vi "Main.vi"() -> ()   [LabVIEW 2020]
doc: "This template is for the Queued Message Handler design pattern.\n\nThe Event Handling Loop generates messages based on user interface actions.\n\nThe Message Handling Loop processes messages generated by the Event Handling Loop, or by other messages. The messages are string values, so new messages can be added easily to the Message Cases case structure in the Message Handling Loop. Each message cluster can also provide an optional value for Message Data, which is a variant that can be converted to whatever message-specific data is required."
uses:
  <vilib>/ErrorRing/Error Ring.xnode
  controls/oled UI Data.ctl
  support/Message Queue/oled Message Queue.lvlib
  support/User Event - Stop/oled User Event - Stop.lvlib
  support/Message Queue/Enqueue Message (Single).vi
  controls/HL Acq Data.ctl
  controls/Acquisition data --typedef.ctl
  controls/Graph data --typedef.ctl
  <vilib>/Utility/error.llb/Error Cluster From Error Code.vi
  <vilib>/DAQmx/read.llb/DAQmx Read (Analog DBL 1Chan 1Samp).vi
  <vilib>/Instr/_visa.llb/VISA Configure Serial Port (Instr).vi
  <vilib>/DAQmx/create/channels.llb/DAQmx Create Channel (AI-Voltage-Basic).vi
  support/Message Queue/Enqueue Message (Array).vi
  controls/Color --typedef.ctl
panel:
  in  "Color":T1 caption="Color de emisión"
  in  "Inicio de Barrido (V)":dbl
  out "Status":string
  in  "milliseconds to wait":i32=200
  out "Eff L-V":cluster{dbl[], dbl[]}(graph) caption="L-V"
  out "EFf I-V":cluster{dbl[], dbl[]}(graph) caption="L-V"
  in  "Puerto serial Fuente":refnum<visa-resource-name>="COM1"
  out "J-V":cluster{dbl[], dbl[]}(graph)
  out "L-V":cluster{dbl[], dbl[]}(graph)
  in  "OLED A":dbl=0.07 caption="Area del OLED [cm2]"
  in  "OLED-PD dist":dbl=1.0 caption="Distancia OLED-fotodiodo [cm]"
  in  "Protection C":dbl=0.1 caption="Corriente de Proteccion [A]\n(0.1-0.3A recomendado)"
  in  "Max V":dbl=2.0 caption="Voltaje máximo [V]\n(20V max. recomendado)"
  in  "Iniciar":bool
  in  "Step #":dbl=100.0 caption="Numero de pasos\n(100-250 recomendado)"
  in  "Exit":bool
  # "Sistema de caracterización de OLEDs"
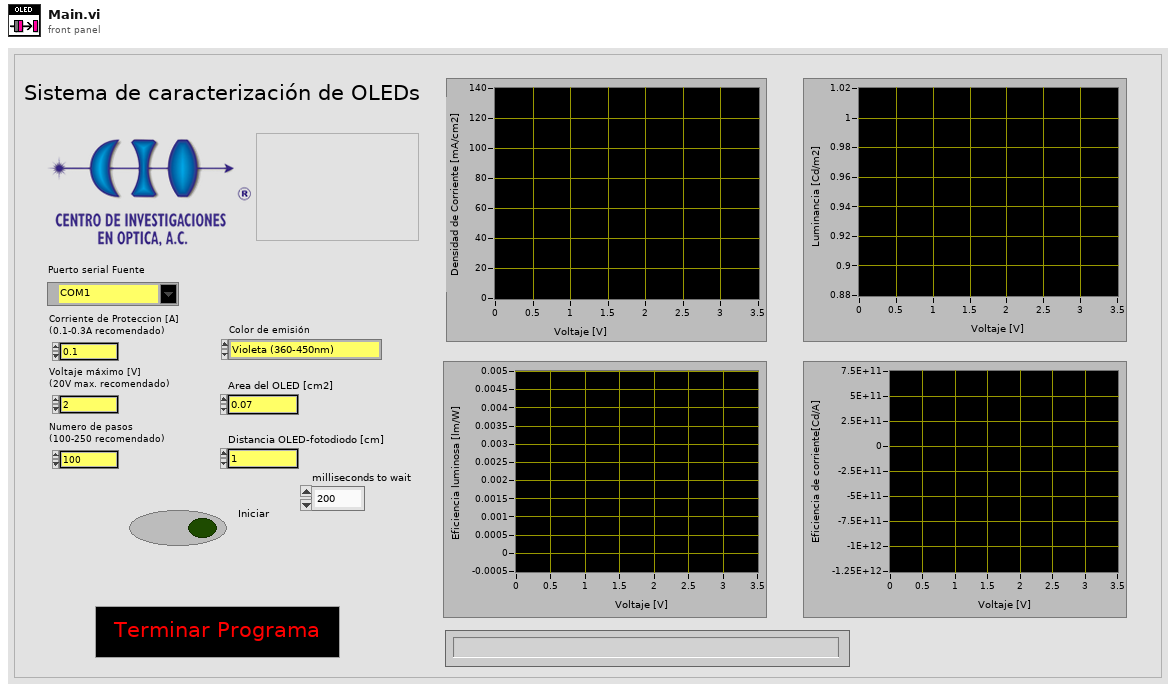
[diagram p1: front panel]
types:
  T1 = typedef "Color --typedef.ctl" = enum16{"Violeta (360-450nm)", "Azul (450-500nm)", "Verde(500-570nm)", "Amarillo (570-590nm)", "Naranja (600-610nm)", "Rojo (610-670nm)", "Blanco"}
  T2 = typedef "oled UI Data.ctl" = cluster{"Status":string, "Puerto serial":refnum<visa-resource-name>, "AI task":refnum<k21>, "Protection C":dbl, "Sweep start V":dbl, "Max V":dbl, "delta V":dbl, "Graph data":T3}
  T3 = typedef "Graph data --typedef.ctl" = cluster{"Voltaje [V]":dbl[], "Corriente [mA]":dbl[], "Densidad de corriente [CD/A]":dbl[], "Iluminancia [Lm/m2]":dbl[], "Luminance [Cd/m2]":dbl[], "Ef corriente [Cd/A]":dbl[], "Ef Luminosa [Cd/W]":dbl[], "V detector [V]":dbl[], "Pin [W]":dbl[]}
  T4 = cluster{"User event - Stop":refnum<user-event>, "User event - Sleep HL":refnum<user-event>, "User event -  Wake HL":refnum<user-event>}
  T5 = typedef "oled Message Queue.lvlib/All Message Queues.ctl" = cluster{"UI":refnum<queue>}
  T6 = typedef "HL Acq Data.ctl" = cluster{"dV":dbl, "Vmax":dbl, "Vo":dbl}
  T7 = typedef "Acquisition data --typedef.ctl" = cluster{"Iluminancia  lm/m2":dbl, "DAQ AV":dbl, "Luminancia (Cd/m2)":dbl, "Pin(W)":dbl, "SM V":dbl, "SM I":dbl, "OLED Area cm2":dbl}
  T8 = cluster{"Voltaje [V]":dbl[], "Luminance [Cd/m2]":dbl[]}
  T9 = cluster{"Voltaje [V]":dbl[], "V detector [V]":dbl[]}
  T10 = cluster{"Voltaje [V]":dbl[], "Ef corriente [Cd/A]":dbl[]}
  T11 = cluster{"Voltaje [V]":dbl[], "Corriente [mA]":dbl[]}
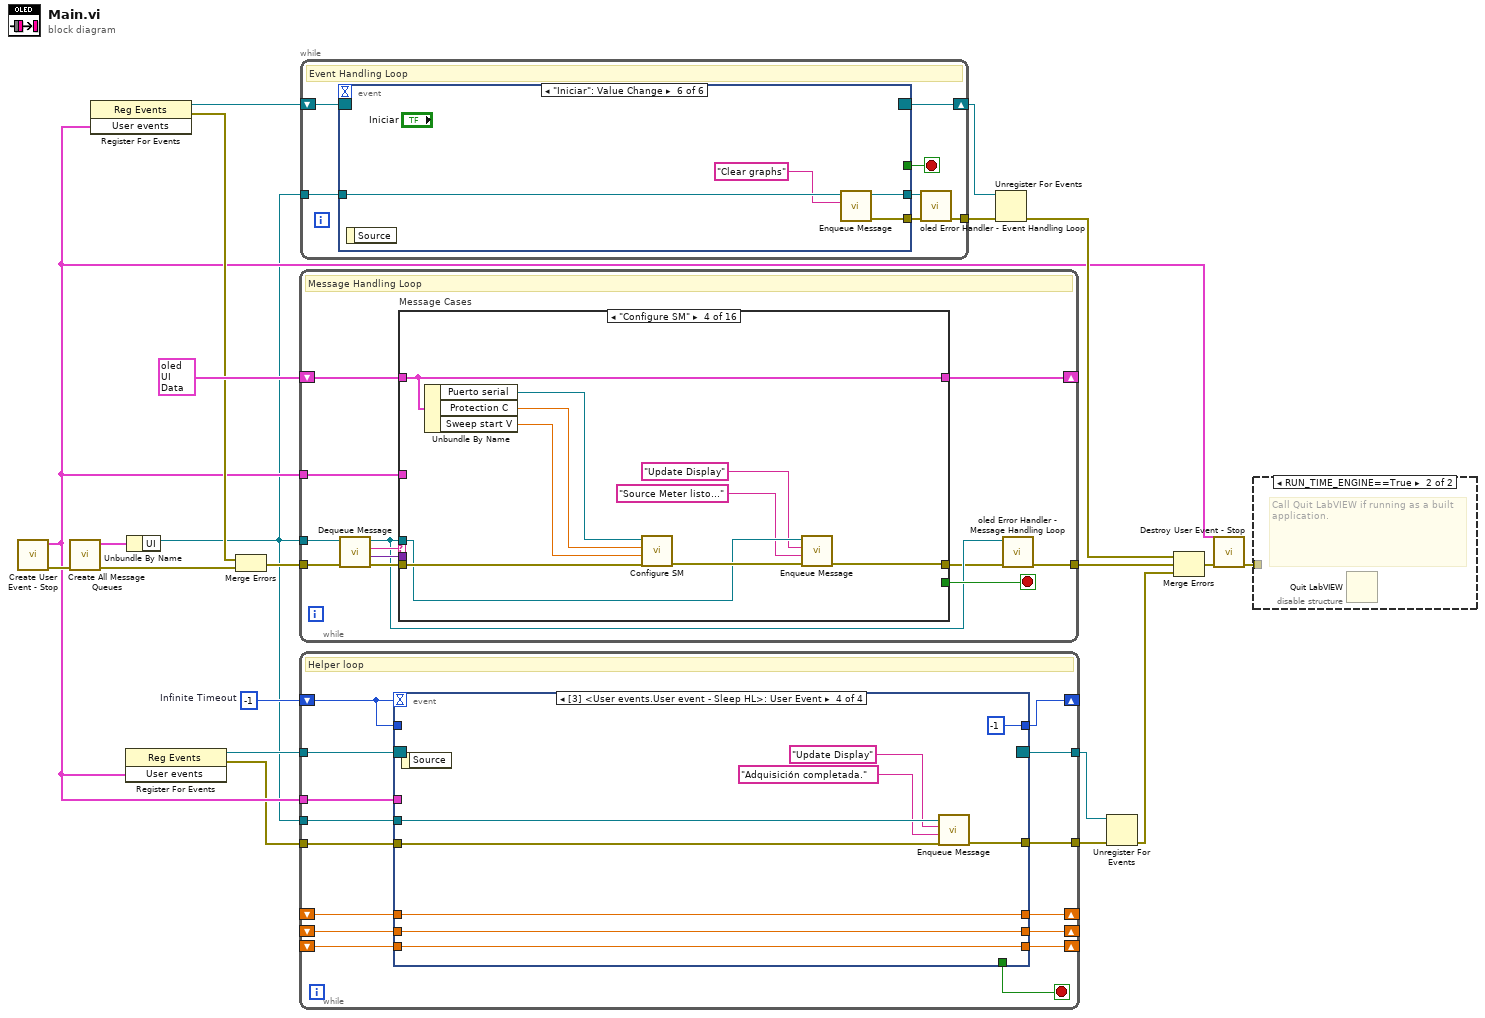
[diagram p0: block diagram]
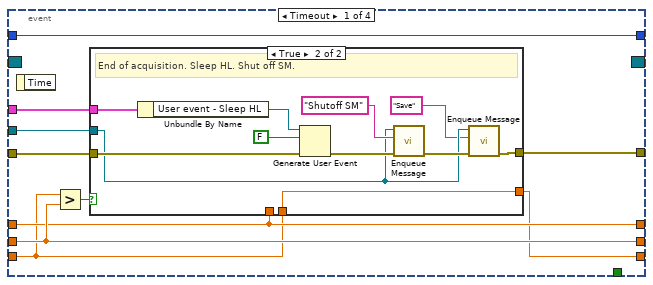
[diagram p2: hidden frame]
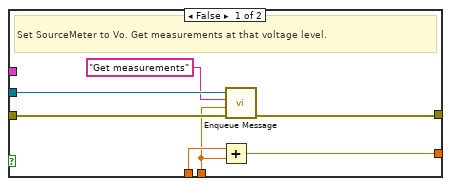
[diagram p3: hidden frame]
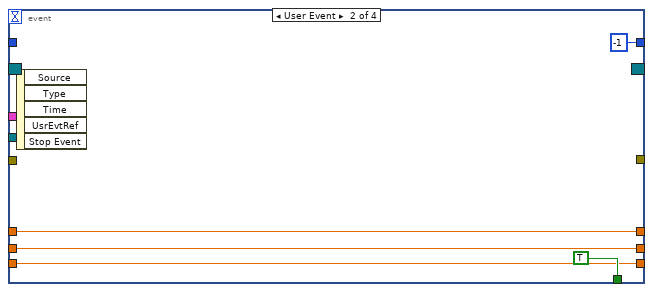
[diagram p4: hidden frame]
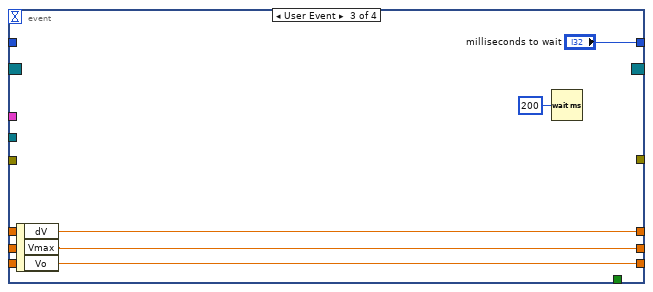
[diagram p5: hidden frame]
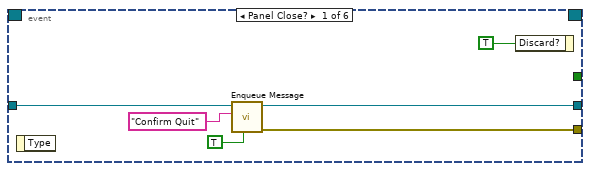
[diagram p6: hidden frame]
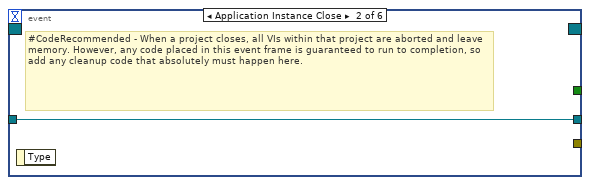
[diagram p7: hidden frame]
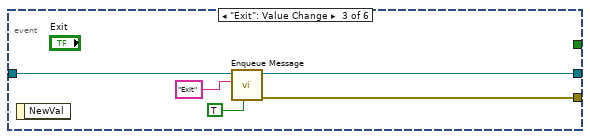
[diagram p8: hidden frame]
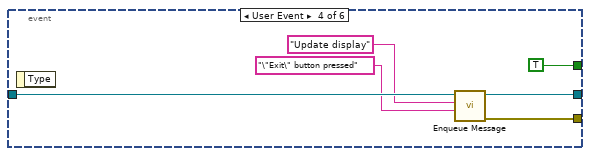
[diagram p9: hidden frame]
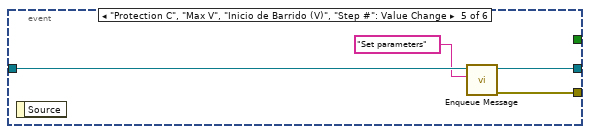
[diagram p10: hidden frame]
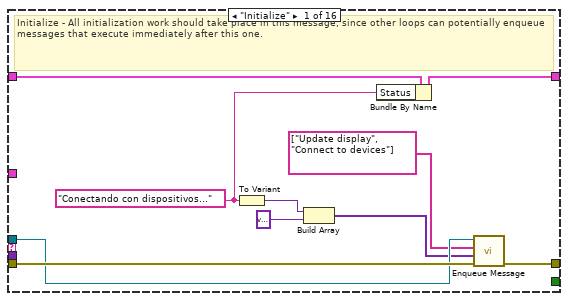
[diagram p11: hidden frame]
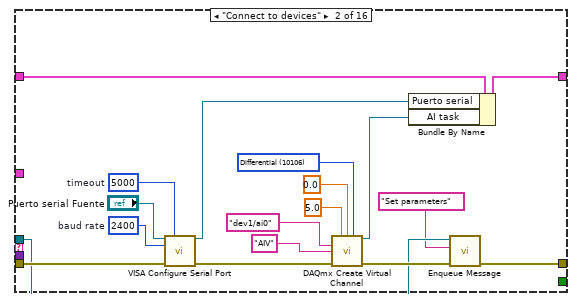
[diagram p12: hidden frame]
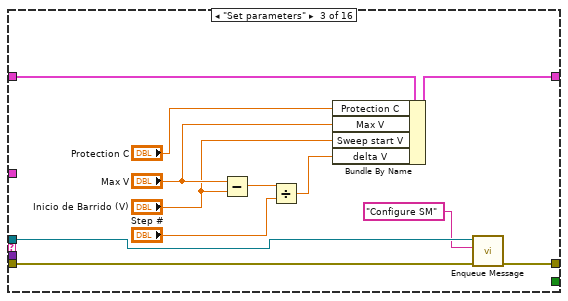
[diagram p13: hidden frame]
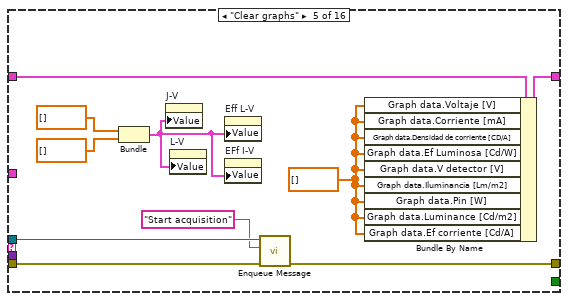
[diagram p14: hidden frame]
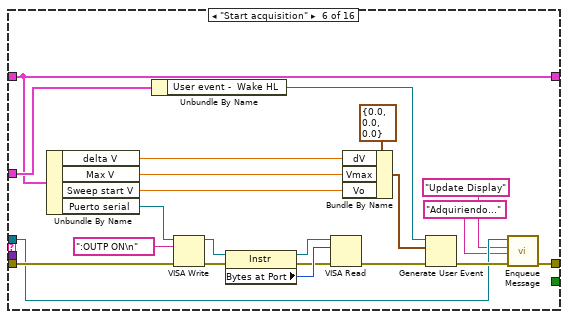
[diagram p15: hidden frame]
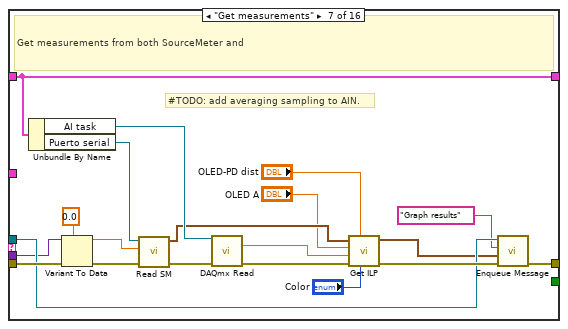
[diagram p16: hidden frame]
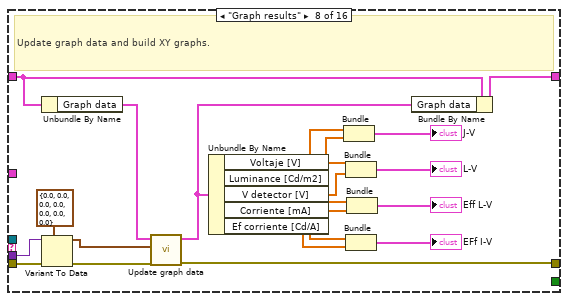
[diagram p17: hidden frame]
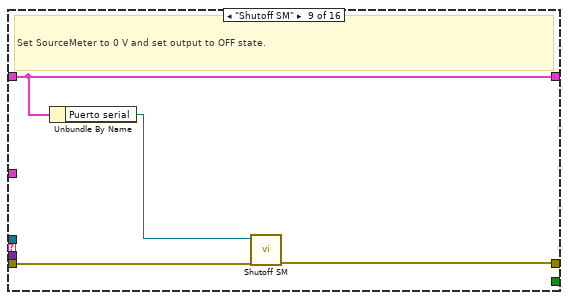
[diagram p18: hidden frame]
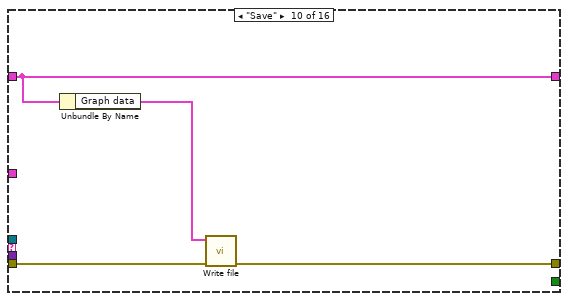
[diagram p19: hidden frame]
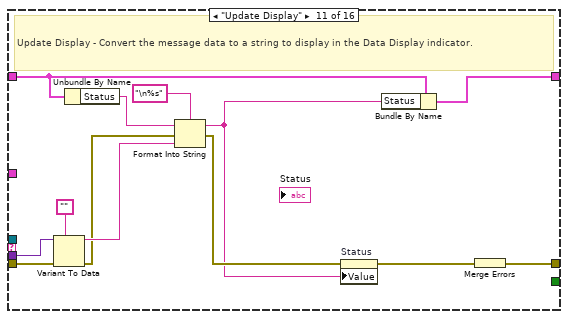
[diagram p20: hidden frame]
diagram:
  w9 = -1  # Infinite Timeout
  n1 = call "Create User Event - Stop.vi"() -> ("error out"=w19:errorcluster, "User events"=w4:T4)  [unwired: 10 in]
  n2 = call "Create All Message Queues.vi"("error in (no error)"=w19) -> ("error out"=w21:errorcluster, "Message Queues out"=w20:T5)  [unwired: 9 in]
  n3 = register-events(w4) -> (reference out=w12:refnum<event-registration>, error out=w10:errorcluster)  [unwired: 2 in]
  n4 = register-events(w4) -> (reference out=w8:refnum<event-registration>, error out=w2:errorcluster)  [unwired: 2 in]
  n5 = Unbundle By Name(w20) -> ("UI"=w1:refnum<queue>)
  n6 = Merge Errors(w10, w21) -> (w11:errorcluster)
  n7 = while {
    tunnel: w1 -> [w25]
    shift-right: [w32] -> _
    shift-left: T2 {"Status"="", "Puerto serial"="", "AI task"="", "Protection C"=0.0, "Sweep start V"=0.0, "Max V"=0.0, "delta V"=0.0, "Graph data"={"Voltaje [V]"=[], "Corriente [mA]"=[], "Densidad de corriente [CD/A]"=[], "Iluminancia [Lm/m2]"=[], "Luminance [Cd/m2]"=[], "Ef corriente [Cd/A]"=[], "Ef Luminosa [Cd/W]"=[], "V detector [V]"=[], "Pin [W]"=[]}} ("Data Cluster") -> [w33]
    tunnel: w4 -> [w30]
    tunnel: w11 -> [w29]
    tunnel: [w23] -> w6
    stop <- w31 stop-if-true
    # "Message Handling Loop"
    n8 = call "Dequeue Message.vi"("error in (no error)"=w29, "Message Queue"=w25) -> ("error out"=w28:errorcluster, "Message Data"=w26:variant, "Message"=w27:string, "dup Message Queue"=w24:refnum<queue>)  [unwired: 6 in]
    n9 = case "Message Cases" shown="\"Configure SM\"" w27 {
      selector: w27 -> [_ _ _ _ _ _ _ _ _ _ _ _ _ _ _ w223]
      tunnel: w24 -> [w39 w45 w63 w76 w85 w104 w127 _ _ _ _ w176 w192 _ w222 _]
      tunnel: w28 -> [w42 w61 w65 w79 w87 w110 w135 w154 w158 w160 w174 w184 w196 w199 w216 _]
      tunnel: [w43 w46 w64 w77 w86 w105 w128 w146 w157 w159 w175 w179 w194 w197 w219 w224] -> w22
      tunnel: w33 -> [w41 w57 w72 w83 w88 w108 w134 w149 w156 w162 w165 w183 w195 w198 w212 w225]
      tunnel: [w40 w55 w67 w83 w90 w108 w134 w148 w156 w162 w163 w183 w195 w198 w212 w225] -> w32
      tunnel: [_ _ _ _ _ _ _ _ _ _ _ _ _ _ TRUE _] -> w31
      tunnel: w26 -> [_ _ _ _ _ _ w118 w152 _ _ w173 w182 _ _ w213 _]
      tunnel: w30 -> [_ _ _ _ _ w111 _ _ _ _ _ _ _ _ w218 _]
      frame "Initialize" {
        w34 = "Conectando con dispositivos..." ("Initial Message")
        # "Initialize - All initialization work should take place in this message, since other loops can potentially enqueue messages that execute immediately after this one."
        n10 = To Variant(anything=w34) -> (Variant=w37:variant)
        n11 = Build Array(w37, variant ("element")) -> (w35:variant[])
        n12 = Bundle By Name(cluster=w41, "Status"=w34) -> (w40:T2)
        n13 = call-poly "Enqueue Message.vi"("error in (no error)"=w42, "Message Data Array"=w35, "Message Array"=string[] ["Update display", "Connect to devices"] ("Message"), "Message Queue"=w39) -> ("error out"=w43:errorcluster)  [unwired: 6 in, 1 out]
      }
      frame "Connect to devices" {
        w49 = 10106 items=["Default"=-1, "RSE"=10083, "NRSE"=10078, "Differential"=10106, "Pseudodifferential"=12529] ("input terminal configuration")
        w58 = u32 5000  # timeout
        w59 = u32 2400  # baud rate
        n14 = call-poly "VISA Configure Serial Port"("VISA resource name"="Puerto serial Fuente", "timeout (10sec)"=w58, "baud rate (9600)"=w59, "error in (no error)"=w61) -> ("VISA resource name out"=w56:refnum<visa-resource-name>, "error out"=w54:errorcluster)  [unwired: 3 in, 7 out]
        n15 = call-poly <vilib>:"DAQmx Create Virtual Channel.vi"("maximum value"=5.0, "minimum value"=0.0, "input terminal configuration"=w49, "physical channels"="dev1/ai0", "name to assign"="AIV", "error in"=w54) -> ("task out"=w48:refnum<k21>, "error out"=w47:errorcluster)  [unwired: 8 in]
        n16 = Bundle By Name(cluster=w57, "Puerto serial"=w56, "AI task"=w48) -> (w55:T2)
        n17 = call-poly "Enqueue Message.vi"("error in (no error)"=w47, "Message"="Set parameters", "Message Queue"=w45) -> ("error out"=w46:errorcluster)  [unwired: 7 in, 1 out]
      }
      frame "Set parameters" {
        n18 = Subtract(x="Max V", y="Inicio de Barrido (V)") -> (x-y=w73:dbl)
        n19 = Divide(x=w73, y="Step #") -> (x/y=w68:dbl)
        n20 = Bundle By Name(cluster=w72, "Protection C"="Protection C", "Max V"="Max V", "Sweep start V"="Inicio de Barrido (V)", "delta V"=w68) -> (w67:T2)
        n21 = call-poly "Enqueue Message.vi"("error in (no error)"=w65, "Message"="Configure SM", "Message Queue"=w63) -> ("error out"=w64:errorcluster)  [unwired: 7 in, 1 out]
      }
      frame "Configure SM" {
        n22 = Unbundle By Name(w83) -> ("Puerto serial"=w81:refnum<visa-resource-name>, "Protection C"=w80:dbl, "Sweep start V"=w82:dbl)
        n23 = call "Configure SM.vi"("error in (no error)"=w79, "Sweep start V"=w82, "Protection C"=w80, "Puerto serial"=w81) -> ("error out"=w78:errorcluster)  [unwired: 7 in]
        n24 = call-poly "Enqueue Message.vi"("error in (no error)"=w78, "Message Data"="Source Meter listo..." ("Message"), "Message"="Update Display", "Message Queue"=w76) -> ("error out"=w77:errorcluster)  [unwired: 6 in, 1 out]
      }
      frame "Clear graphs" {
        w89 = dbl[] []
        n25 = Bundle(dbl[] [], dbl[] []) -> (w91:cluster{dbl[], dbl[]})  [unwired: 1 out]
        n26 = property on="J-V" class="XYGraph (strict)"("Value"=w91) -> ()  [unwired: 2 in, 2 out]
        n27 = property on="L-V" class="XYGraph (strict)"("Value"=w91) -> ()  [unwired: 2 in, 2 out]
        n28 = property on="Eff L-V" class="XYGraph (strict)"("Value"=w91) -> ()  [unwired: 2 in, 2 out]
        n29 = property on="EFf I-V" class="XYGraph (strict)"("Value"=w91) -> ()  [unwired: 2 in, 2 out]
        n30 = call-poly "Enqueue Message.vi"("error in (no error)"=w87, "Message"="Start acquisition", "Message Queue"=w85) -> ("error out"=w86:errorcluster)  [unwired: 7 in, 1 out]
        n31 = Bundle By Name(cluster=w88, "Graph data.Voltaje [V]"=w89, "Graph data.Corriente [mA]"=w89, "Graph data.Densidad de corriente [CD/A]"=w89, "Graph data.Ef Luminosa [Cd/W]"=w89, "Graph data.V detector [V]"=w89, "Graph data.Iluminancia [Lm/m2]"=w89, "Graph data.Pin [W]"=w89, "Graph data.Luminance [Cd/m2]"=w89, "Graph data.Ef corriente [Cd/A]"=w89) -> (w90:T2)
      }
      frame "Start acquisition" {
        n32 = Unbundle By Name(w108) -> ("delta V"=w107:dbl, "Max V"=w113:dbl, "Sweep start V"=w112:dbl, "Puerto serial"=w100:refnum<visa-resource-name>)
        n33 = Unbundle By Name(w111) -> ("User event -  Wake HL"=w109:refnum<user-event>)
        n34 = VISA Write(VISA resource name=w100, write buffer=":OUTP ON\n" ("Comando"), error in (no error)=w110) -> (VISA resource name out=w98:refnum<visa-resource-name>, error out=w95:errorcluster)  [unwired: 1 out]
        n35 = property class="Instr"(reference=w98, error in=w95) -> (reference out=w97:refnum<visa-resource-name>, error out=w94:errorcluster, "Bytes at Port"=w96:u32)
        n36 = VISA Read(VISA resource name=w97, byte count=w96, error in (no error)=w94) -> (error out=w99:errorcluster)  [unwired: 3 out]
        n37 = Bundle By Name(cluster=T6 {"dV"=0.0, "Vmax"=0.0, "Vo"=0.0} ("event data"), "dV"=w107, "Vmax"=w113, "Vo"=w112) -> (w114:T6)
        n38 = Generate User Event(user event=w109, event data cluster=w114, error in=w99) -> (error out=w106:errorcluster)  [unwired: 1 in, 1 out]
        n39 = call-poly "Enqueue Message.vi"("error in (no error)"=w106, "Message Data"="Adquiriendo..." ("Message"), "Message"="Update Display", "Message Queue"=w104) -> ("error out"=w105:errorcluster)  [unwired: 6 in, 1 out]
      }
      frame "Get measurements" {
        # "#TODO: add averaging sampling to AIN."
        # "Get measurements from both SourceMeter and"
        n40 = Unbundle By Name(w134) -> ("AI task"=w131:refnum<k21>, "Puerto serial"=w133:refnum<visa-resource-name>)
        n41 = Variant To Data(error in=w135, type=0.0, Variant=w118) -> (data=w117:dbl, error out=w120:errorcluster)
        n42 = call "Read SM.vi"("error in (no error)"=w120, "Vo"=w117, "Puerto serial"=w133) -> ("error out"=w132:errorcluster, "Acquistion Data"=w124:T7)  [unwired: 7 in]
        n43 = call-poly <vilib>:"DAQmx Read.vi"("task/channels in"=w131, "error in"=w132) -> ("data"=w123:dbl, "error out"=w130:errorcluster)  [unwired: 11 in, 1 out]
        n44 = call "Get ILP.vi"("Color"="Color", "OLED-PD dist"="OLED-PD dist", "error in (no error)"=w130, "DAQ V"=w123, "OLED A"="OLED A", "Acquistion Data"=w124) -> ("error out"=w129:errorcluster, "Acquistion Data"=w125:T7)  [unwired: 4 in]
        n45 = call-poly "Enqueue Message.vi"("error in (no error)"=w129, "Message Data"=w125, "Message"="Graph results", "Message Queue"=w127) -> ("error out"=w128:errorcluster)  [unwired: 6 in, 1 out]
      }
      frame "Graph results" {
        # "Update graph data and build XY graphs."
        n46 = Unbundle By Name(w149) -> ("Graph data"=w150:T3)
        n47 = Variant To Data(error in=w154, type=T7 {"Iluminancia  lm/m2"=0.0, "DAQ AV"=0.0, "Luminancia (Cd/m2)"=0.0, "Pin(W)"=0.0, "SM V"=0.0, "SM I"=0.0, "OLED Area cm2"=0.0} ("output cluster"), Variant=w152) -> (data=w151:T7, error out=w147:errorcluster)
        n48 = call "Update graph data.vi"("error in (no error)"=w147, "Acquisition data"=w151, "Graph data"=w150) -> ("error out"=w146:errorcluster, "Graph data"=w140:T3)  [unwired: 7 in]
        n49 = Unbundle By Name(w140) -> ("Voltaje [V]"=w139:dbl[], "Luminance [Cd/m2]"=w145:dbl[], "V detector [V]"=w138:dbl[], "Corriente [mA]"=w137:dbl[], "Ef corriente [Cd/A]"=w136:dbl[])
        n50 = Bundle("Voltaje [V]"=w139, "Luminance [Cd/m2]"=w145) -> (→"J-V":T8)  [unwired: 1 in]
        n51 = Bundle("Voltaje [V]"=w139, "V detector [V]"=w138) -> (→"L-V":T9)  [unwired: 1 in]
        n52 = Bundle("Voltaje [V]"=w139, "Ef corriente [Cd/A]"=w136) -> (→"EFf I-V":T10)  [unwired: 1 in]
        n53 = Bundle("Voltaje [V]"=w139, "Corriente [mA]"=w137) -> (→"Eff L-V":T11)  [unwired: 1 in]
        n54 = Bundle By Name(cluster=w149, "Graph data"=w140) -> (w148:T2)
      }
      frame "Shutoff SM" {
        # "Set SourceMeter to 0 V and set output to OFF state."
        n55 = Unbundle By Name(w156) -> ("Puerto serial"=w155:refnum<visa-resource-name>)
        n56 = call "Shutoff SM.vi"("error in (no error)"=w158, "Puerto serial"=w155) -> ("error out"=w157:errorcluster)  [unwired: 8 in, 1 out]
      }
      frame "Save" {
        n57 = Unbundle By Name(w162) -> ("Graph data"=w161:T3)
        n58 = call "Write file.vi"("error in (no error)"=w160, "Graph data"=w161) -> ("error out"=w159:errorcluster)  [unwired: 9 in]
      }
      frame "Update Display" {
        # "Update Display - Convert the message data to a string to display in the Data Display indicator."
        n59 = Variant To Data(error in=w174, type="", Variant=w173) -> (data=w169:string, error out=w167:errorcluster)
        n60 = Unbundle By Name(w165) -> ("Status"=w171:string)
        n61 = Format Into String(format string="\n%s", initial string=w171, error in=w167, w169) -> (resulting string=w164:string, error out=w166:errorcluster)
        n62 = property on="Status" class="Str"(error in=w166, "Value"=w164) -> (error out=w168:errorcluster)  [unwired: 1 in, 1 out]
        n63 = Bundle By Name(cluster=w165, "Status"=w164) -> (w163:T2)
        n64 = Merge Errors(w168) -> (w175:errorcluster)
      }
      frame "Error" {
        # "Error - Display an error dialog. This message is sent by the \"Error Handler\" VIs at the end of other loops in this application."
        n65 = Variant To Data(error in=w184, type=errorcluster {"status"=FALSE, "code"=0, "source"=""} ("error constant"), Variant=w182) -> (data=w178:errorcluster, error out=w180:errorcluster)
        n66 = case shown="Default" w178 {
          selector: w178 -> [_ w186]
          tunnel: [_ w185] -> w177
          tunnel: w176 -> [_ _]
          frame No Error {
          }
          frame Default {
            n67 = Unbundle By Name(w186) -> ("code"=w188:i32)
            n68 = call "oled Error logger.vi"("error in (no error)"=w186) -> ("error out"=w185:errorcluster)  [unwired: 10 in]
            n69 = Format Into String(format string="Error desconocido. Código de error: %d. ", w188) -> (resulting string=w187:string)  [unwired: 2 in, 1 out]
            n70 = One Button Dialog(message=w187) -> ()  [unwired: 1 in, 1 out]
          }
        }
        n71 = Merge Errors(w180, w177) -> (w179:errorcluster)
      }
      frame "Confirm Quit" {
        # "#CodeNeeded - If you want to provide an \"Are you sure\" dialog (or some other notification) before the application exits, place that code here. This message is typically sent from a Panel Close? event."
        # "Confirm Quit - Message that can confirm whether or not the user wants to exit the application."
        n72 = call-poly "Enqueue Message.vi"("Priority Message? (F)"=TRUE, "error in (no error)"=w196, "Message"="Exit", "Message Queue"=w192) -> ("error out"=w193:errorcluster)  [unwired: 6 in, 1 out]
        n73 = Merge Errors(w193) -> (w194:errorcluster)
      }
      frame "---Copy This Frame---" {
        # "Duplicate this frame when creating new messages.  Change this comment in the duplicated frame to describe this message."
        n74 = Merge Errors(w199) -> (w197:errorcluster)
      }
      frame "Exit" {
        # "Stop the VI"
        # "Release the message queue reference"
        # "Close communicastion, stop AI task and exit application."
        n75 = Unbundle By Name(w212) -> ("Puerto serial"=w206:refnum<visa-resource-name>, "AI task"=w211:refnum<k21>)
        n76 = Variant To Data(type=errorcluster {"status"=FALSE, "code"=0, "source"=""} ("error constant"), Variant=w213) -> (data=w214:errorcluster)  [unwired: 1 in, 1 out]
        n77 = call <vilib>:"Simple Error Handler.vi"("error in (no error)"=w214) -> ()  [unwired: 4 in, 5 out]
        n78 = Unbundle By Name(w218) -> ("User event - Stop"=w204:refnum<user-event>)
        n79 = call "Shutoff SM.vi"("Puerto serial"=w206) -> ("error out"=w205:errorcluster, "Puerto serial"=w202:refnum<visa-resource-name>)  [unwired: 9 in]
        n80 = call <vilib>:"DAQmx Stop Task.vi"("task/channels in"=w211) -> ("task out"=w210:refnum<k21>, "error out"=w209:errorcluster)  [unwired: 13 in]
        n81 = Release Queue(queue=w222, error in (no error)=w216) -> (error out=w220:errorcluster)  [unwired: 1 in, 2 out]
        n82 = call <vilib>:"DAQmx Clear Task.vi"("task in"=w210, "error in"=w209) -> ("error out"=w207:errorcluster)  [unwired: 13 in]
        n83 = VISA Write(VISA resource name=w202, write buffer=":SYST:RSEN OFF\n" ("Comando"), error in (no error)=w205) -> (VISA resource name out=w201:refnum<visa-resource-name>, error out=w203:errorcluster)  [unwired: 1 out]
        n84 = VISA Close(VISA resource name=w201, error in (no error)=w203) -> (error out=w208:errorcluster)
        n85 = call "Fire User Event - Stop.vi"("User Event - Stop"=w204) -> ("error out"=w217:errorcluster)  [unwired: 10 in]
        n86 = Merge Errors(w217, w220, w208, w207) -> (w219:errorcluster)
      }
      frame Default {
        # "'Default' case only runs if there is a message that isn't defined in any of the other cases.  Output a programming error."
        n87 = xnode "Error Ring"("parameter 0"=w223) -> ("error out"=w224:errorcluster)
      }
    }
    n88 = call "oled Error Handler - Message Handling Loop.vi"("error in (no error)"=w22, "Message Queue"=w24) -> ("dup error in"=w23:errorcluster)  [unwired: 8 in, 1 out]
  }
  n89 = while {
    shift-right: [w245] -> _
    shift-left: w9 -> [w244]
    tunnel: w8 -> [w247]
    tunnel: [w243] -> w7
    shift-right: [w242] -> _
    shift-left: _ -> [w239]
    shift-right: [w241] -> _
    shift-left: _ -> [w238]
    shift-right: [w240] -> _
    shift-left: _ -> [w237]
    tunnel: w4 -> [w236]
    tunnel: [w235] -> w3
    tunnel: w2 -> [w234]
    tunnel: w1 -> [w233]
    stop <- w246 stop-if-true
    # "Helper loop"
    n90 = event shown="[3] <User events.User event - Sleep HL>: User Event" {
      selector: w247 -> [_ _ _ _]
      dyn-events: [_ _ _ _] -> w243
      timeout: w244 -> [_ _ _ _]
      tunnel: [_ TRUE _ _] -> w246
      tunnel: w244 -> [w257 _ _ _]
      tunnel: [w257 -1 ("Infinite Timeout") "milliseconds to wait" -1 ("Infinite Timeout")] -> w245
      tunnel: [w251 w278 w285 w293] -> w242
      tunnel: [w255 w277 w284 w292] -> w241
      tunnel: [w249 w276 w283 w291] -> w240
      tunnel: w239 -> [w251 w278 _ w293]
      tunnel: w238 -> [w255 w277 _ w292]
      tunnel: w237 -> [w250 w276 _ w291]
      tunnel: w236 -> [w254 _ _ _]
      tunnel: [w253 _ _ w290] -> w235
      tunnel: w234 -> [w252 _ _ w288]
      tunnel: w233 -> [w248 _ _ w289]
      event Timeout {
        n91 = event-data() -> ()  [unwired: 1 in, 1 out]
        n92 = Greater?(x=w250, y=w255) -> (0:w256:bool)
        n93 = case shown="True" w256 {
          tunnel: w254 -> [_ w275]
          tunnel: [w261 w267] -> w253
          tunnel: w252 -> [w262 w272]
          tunnel: w251 -> [w264 _]
          tunnel: w250 -> [w258 w271]
          tunnel: [w263 w271] -> w249
          tunnel: w248 -> [w260 w266]
          frame False {
            # "Set SourceMeter to Vo. Get measurements at that voltage level."
            n94 = Add(x=w264, y=w258) -> (x+y=w263:dbl)
            n95 = call-poly "Enqueue Message.vi"("error in (no error)"=w262, "Message Data"=w258, "Message"="Get measurements", "Message Queue"=w260) -> ("error out"=w261:errorcluster)  [unwired: 6 in, 1 out]
          }
          frame True {
            # "End of acquisition. Sleep HL. Shut off SM."
            n96 = Unbundle By Name(w275) -> ("User event - Sleep HL"=w274:refnum<user-event>)
            n97 = Generate User Event(user event=w274, event data cluster=FALSE ("event data"), error in=w272) -> (error out=w270:errorcluster)  [unwired: 1 in, 1 out]
            n98 = call-poly "Enqueue Message.vi"("error in (no error)"=w270, "Message"="Shutoff SM", "Message Queue"=w266) -> ("error out"=w268:errorcluster)  [unwired: 7 in, 1 out]
            n99 = call-poly "Enqueue Message.vi"("error in (no error)"=w268, "Message"="Save", "Message Queue"=w266) -> ("error out"=w267:errorcluster)  [unwired: 7 in, 1 out]
          }
        }
      }
      event User Event {
        n100 = event-data() -> ()  [unwired: 1 in, 5 out]
      }
      event User Event {
        n101 = event-data() -> ("dV"=w285:dbl, "Vmax"=w284:dbl, "Vo"=w283:dbl)  [unwired: 1 in]
        n102 = Wait (ms)(milliseconds to wait=u32 200) -> ()  [unwired: 1 out]
      }
      event User Event {
        n103 = event-data() -> ()  [unwired: 1 in, 1 out]
        n104 = call-poly "Enqueue Message.vi"("error in (no error)"=w288, "Message Data"="Adquisición completada." ("Message"), "Message"="Update Display", "Message Queue"=w289) -> ("error out"=w290:errorcluster)  [unwired: 6 in, 1 out]
      }
    }
  }
  n105 = while {
    tunnel: w1 -> [w301]
    shift-right: [w299] -> w16
    shift-left: w12 -> [w300]
    tunnel: [w295] -> w13
    stop <- w297 stop-if-true
    # "Event Handling Loop"
    n106 = event shown="[5] \"Iniciar\": Value Change" {
      selector: w300 -> [_ _ _ _ _ _]
      dyn-events: [_ _ _ _ _ _] -> w299
      timeout: _ -> [_ _ _ _ _ _]
      tunnel: [_ _ _ TRUE ("Discard?") _ _] -> w297
      tunnel: w301 -> [w306 w308 w313 w318 w323 w327]
      tunnel: [w305 _ w312 w316 w321 w325] -> w298
      tunnel: [w304 w308 w311 w317 w322 w326] -> w296
      event Panel Close? {
        n107 = event-data() -> ()  [unwired: 1 in, 1 out]
        n108 = call-poly "Enqueue Message.vi"("Priority Message? (F)"=TRUE, "Message"="Confirm Quit", "Message Queue"=w306) -> ("error out"=w305:errorcluster, "dup Message Queue"=w304:refnum<queue>)  [unwired: 7 in]
        n109 = event-data("Discard?"=TRUE) -> ()  [unwired: 1 in, 1 out]
      }
      event Application Instance Close {
        # "#CodeRecommended - When a project closes, all VIs within that project are aborted and leave memory. However, any code placed in this event frame is guaranteed to run to completion, so add any cleanup code that absolutely must happen here."
        n110 = event-data() -> ()  [unwired: 1 in, 1 out]
      }
      event "Exit": Value Change {
        n111 = event-data() -> ()  [unwired: 1 in, 1 out]
        n112 = call-poly "Enqueue Message.vi"("Priority Message? (F)"=TRUE, "Message"="Exit", "Message Queue"=w313) -> ("error out"=w312:errorcluster, "dup Message Queue"=w311:refnum<queue>)  [unwired: 7 in]
      }
      event User Event {
        n113 = event-data() -> ()  [unwired: 1 in, 1 out]
        n114 = call-poly "Enqueue Message.vi"("Message Data"="\"Exit\" button pressed" ("VI Stopped"), "Message"="Update display", "Message Queue"=w318) -> ("error out"=w316:errorcluster, "dup Message Queue"=w317:refnum<queue>)  [unwired: 7 in]
      }
      event "Protection C", "Max V", "Inicio de Barrido (V)", "Step #": Value Change {
        n115 = event-data() -> ()  [unwired: 1 in, 1 out]
        n116 = call-poly "Enqueue Message.vi"("Message"="Set parameters", "Message Queue"=w323) -> ("error out"=w321:errorcluster, "dup Message Queue"=w322:refnum<queue>)  [unwired: 8 in]
      }
      event "Iniciar": Value Change {
        n117 = event-data() -> ()  [unwired: 1 in, 1 out]
        n118 = call-poly "Enqueue Message.vi"("Message"="Clear graphs", "Message Queue"=w327) -> ("error out"=w325:errorcluster, "dup Message Queue"=w326:refnum<queue>)  [unwired: 8 in]
      }
    }
    n119 = call "oled Error Handler - Event Handling Loop.vi"("error in (no error)"=w298, "Message Queue"=w296) -> ("dup error in"=w295:errorcluster)  [unwired: 8 in, 1 out]
  }
  n120 = Unregister For Events(event registration refnum=w16, error in=w13) -> (error out=w17:errorcluster)
  n121 = Unregister For Events(event registration refnum=w7, error in=w3) -> (error out=w5:errorcluster)
  n122 = Merge Errors(w17, w6, w5) -> (w18:errorcluster)
  n123 = call "Destroy User Event - Stop.vi"("error in (no error)"=w18, "User events"=w4) -> ("error out"=w14:errorcluster)  [unwired: 9 in]
  n124 = disable-structure shown="RUN_TIME_ENGINE==True" {
    disable-tunnel: w14 -> [_ _]
    frame condition #0 (active) {
    }
    frame condition #1 {
      # "Call Quit LabVIEW if running as a built application."
      n125 = Quit LabVIEW() -> ()  [unwired: 1 in]
    }
  }
